vi "StateMachine_LIDAR.vi"() -> ()   [LabVIEW 2018]
uses:
  <vilib>/myRIO/Instrument Drivers/Onboard IO/DIO/typedefs/DIO Reference.ctl
  <vilib>/myRIO/Common/Instrument Driver Framework/Utilities/typedefs/myRIO Generic Hardware Reference.ctl
  <vilib>/myRIO/Common/Instrument Driver Framework/Utilities/typedefs/Hardware Version Enum.ctl
  <vilib>/myRIO/Common/Instrument Driver Framework/Utilities/typedefs/myRIO v1.0 Reference.ctl
  <vilib>/myRIO/Common/Instrument Driver Framework/Utilities/typedefs/Generic FPGA Reference.ctl
  <vilib>/myRIO/Common/Instrument Driver Framework/myRIO v1.0/DIO/typedefs/DIO Channels List.ctl
  <vilib>/myRIO/Common/Instrument Driver Framework/myRIO v1.0/DIO/typedefs/DIO Channels Enum.ctl
  <vilib>/userdefined/High Color/nirio_resource_hc.ctl
  enum_data_lidar.ctl
  <vilib>/myRIO/Common/Instrument Driver Framework/Utilities/vis/Is FPGA Ref Available.vi
  <vilib>/myRIO/Common/Instrument Driver Framework/myRIO v1.0/DIO/vis/myRIO v1.1 Open DIO.vi
  <vilib>/myRIO/Instrument Drivers/Onboard IO/DIO/vis/Write.vi
  <vilib>/myRIO/Common/Instrument Driver Framework/Utilities/vis/Validate Channels.vi
  <vilib>/myRIO/Common/Instrument Driver Framework/myRIO v1.0/DIO/vis/myRIO v1.0 Reserve DIO.vi
  <vilib>/myRIO/Common/Instrument Driver Framework/myRIO v1.0/Resource Manager/vis/myRIO v1.0 Reserve Channel List.vi
  <vilib>/myRIO/Common/Instrument Driver Framework/myRIO v1.0/DIO/vis/myRIO v1.0 Build MUX Configuration DIO.vi
  <vilib>/myRIO/Common/Instrument Driver Framework/myRIO v1.0/Resource Manager/vis/myRIO v1.0 Reserve Channel.vi
  <vilib>/myRIO/Common/Instrument Driver Framework/myRIO v1.0/Resource Manager/vis/myRIO v1.0 Unreserve Channel.vi
  <vilib>/myRIO/Common/Instrument Driver Framework/myRIO v1.0/Resource Manager/vis/myRIO v1.0 Create Configuration List.vi
  <vilib>/myRIO/Common/Instrument Driver Framework/myRIO v1.0/Resource Manager/vis/myRIO v1.0 Build Mutex Name.vi
  <vilib>/Utility/VariantDataType/GetNumericInfo.vi
  <vilib>/Utility/error.llb/Error Cluster From Error Code.vi
  <vilib>/myRIO/Common/Instrument Driver Framework/myRIO v1.0/myRIO v1.1 Open.vi
  <vilib>/myRIO/Common/Instrument Driver Framework/Utilities/vis/IO Manager.vi
  <vilib>/myRIO/Common/Instrument Driver Framework/Utilities/vis/Configuration Manager.vi
  <vilib>/myRIO/Common/Instrument Driver Framework/myRIO v1.0/Resource Manager/vis/myRIO v1.0 Configure IO.vi
  <vilib>/myRIO/Common/Instrument Driver Framework/myRIO v1.0/myRIO v1.0 Close.vi
  <vilib>/myRIO/Common/Instrument Driver Framework/myRIO v1.0/DIO/vis/myRIO v1.0 Write DIO.vi
  <vilib>/Instr/_visa.llb/VISA Configure Serial Port (Instr).vi
  <vilib>/myRIO/Express VI/Onboard IO/DO/DO Express VI.xnode
  <vilib>/myRIO/Instrument Drivers/Onboard IO/DIO/vis/myRIO DIO Open.xnode
  <vilib>/myRIO/Instrument Drivers/Onboard IO/DIO/DIO.lvlib
panel:
  out "Graphe XY":cluster{"X":dbl, "Y":dbl}[](graph)
  out "Data":cluster{"Angle":dbl, dbl}[](array[cluster])
  in  "Stop":bool
  out "NbPtsMesure":i32
  out "StartScan OK":bool
  out "Firmware":string
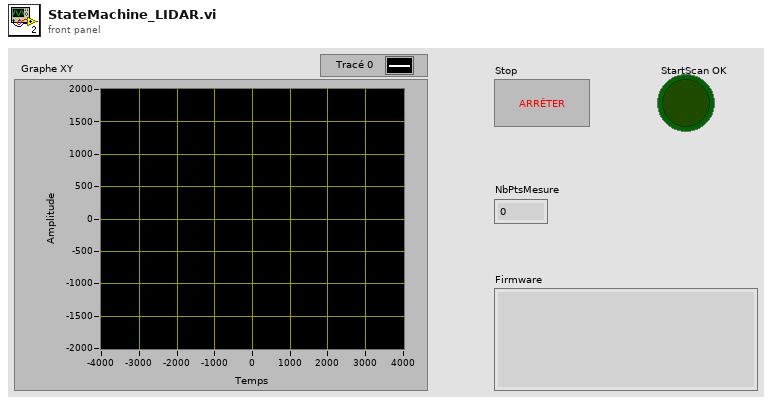
[diagram p1: front panel]
types:
  T1 = typedef "DIO.lvlib/DIO Reference.ctl" = cluster{"myRIO Reference":T2, "DIO Channels List":T6}
  T2 = typedef "myRIO Generic Hardware Reference.ctl" = cluster{"myRIO Model":T3, "myRIO Hardware Reference":T4}
  T3 = typedef "Hardware Version Enum.ctl" = enum16{"Unknown", "myRIO-1900", "myRIO-1950", "roboRIO", "NI ELVIS RIO CM", "ELVIS III"}
  T4 = typedef "myRIO v1.0 Reference.ctl" = cluster{"Generic FPGA Reference":T5, "Allow multiple opens":bool}
  T5 = typedef "Generic FPGA Reference.ctl" = refnum<k20>
  T6 = typedef "DIO Channels List.ctl" = T7[]
  T7 = typedef "DIO Channels Enum.ctl" = enum16{"Not Connected", "C/DIO0", "C/DIO1", "C/DIO2", "C/DIO3", "C/DIO4", "C/DIO5", "C/DIO6", "C/DIO7", "A/DIO0", "A/DIO1", "A/DIO2", "A/DIO3", "A/DIO4", "A/DIO5", "A/DIO6", "A/DIO7", "A/DIO8", "A/DIO9", "A/DIO10", "A/DIO11", "A/DIO12", "A/DIO13", "A/DIO14", "A/DIO15", "A/DIO16", "A/DIO17", "A/DIO18", "A/DIO19", "B/DIO0", "B/DIO1", "B/DIO2", "B/DIO3", "B/DIO4", "B/DIO5", "B/DIO6", "B/DIO7", "B/DIO8", "B/DIO9", "B/DIO10", "B/DIO11", "B/DIO12", "B/DIO13", "B/DIO14", "B/DIO15", "B/DIO16", "B/DIO17", "B/DIO18", "B/DIO19", "LED0", "LED1", "LED2", "LED3", "Button0", "DIO/DIO0", "DIO/DIO1", "DIO/DIO2", "DIO/DIO3", "DIO/DIO4", "DIO/DIO5", "DIO/DIO6", "DIO/DIO7", "DIO/DIO8", "DIO/DIO9", "SPI/CS0", "SPI/CS1", "SPI/CS2", "SPI/CS3", "LED RADIO (Green)", "LED RADIO (Red)", "LED COMM (Green)", "LED COMM (Red)", "LED MODE (Green)", "LED MODE (Red)"}
  T8 = typedef "nirio_resource_hc.ctl" = tag
  T9 = typedef "enum_data_lidar.ctl" = enum16{"Init", "Reset", "Start Scan", "Read Data", "Process Data", "Close"}
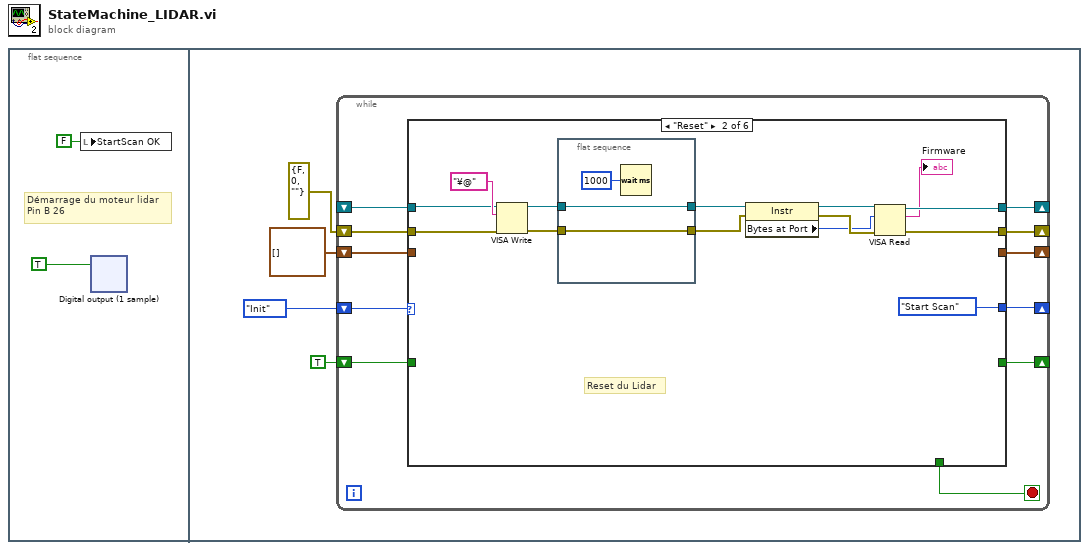
[diagram p0: block diagram]
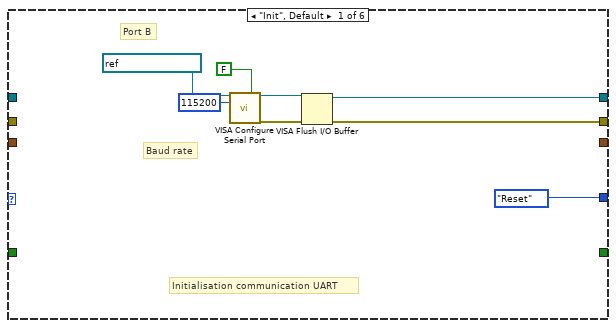
[diagram p2: hidden frame]
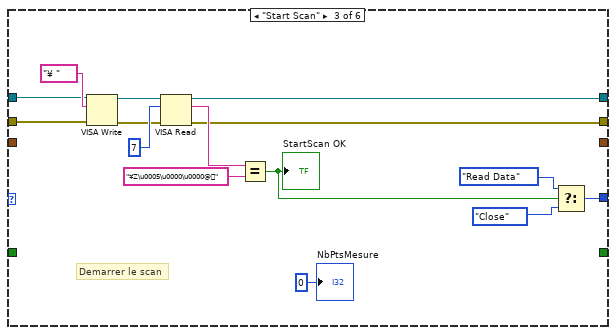
[diagram p3: hidden frame]
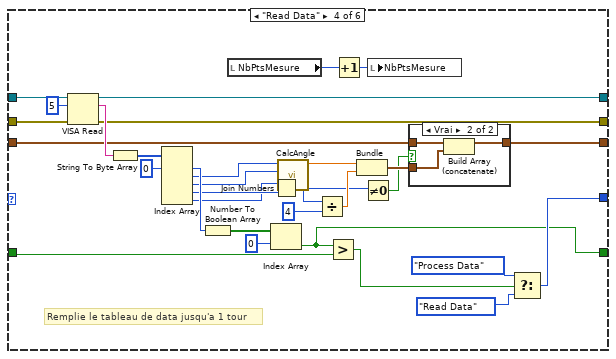
[diagram p4: hidden frame]
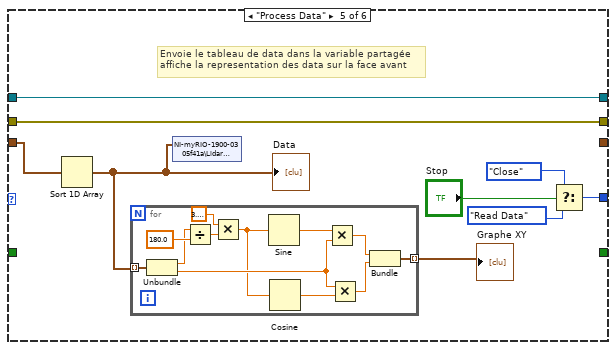
[diagram p6: hidden frame]
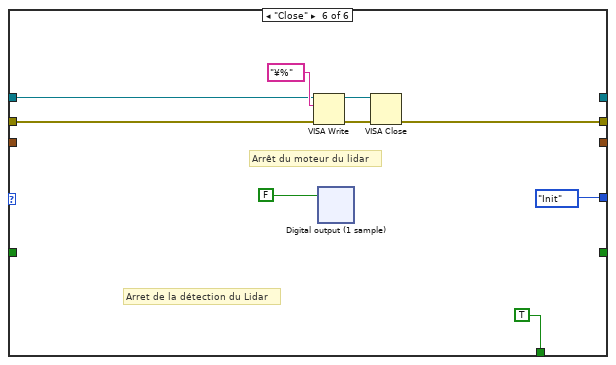
[diagram p7: hidden frame]
diagram:
  n1 = flat-sequence {
    frame #0 {
      # "Démarrage du moteur lidar\nPin B 26"
      n2 = local write "StartScan OK"(FALSE ("StartScan OK")) -> ()
      n3 = xnode "Digital output (1 sample)"("B/DIO13 (Pin 26)"=TRUE) -> ()  [unwired: 1 in, 1 out]
    }
    frame #1 {
      n4 = while {
        shift-right: [w47] -> _
        shift-left: enum_data_lidar."Init" ("Etats") -> [w52]
        shift-right: [w51] -> _
        shift-left: _ -> [w49]
        shift-right: [w50] -> _
        shift-left: errorcluster {"status"=FALSE, "code"=0, "source"=""} ("constante d'erreur") -> [w48]
        shift-right: [w44] -> _
        shift-left: TRUE -> [w45]
        shift-right: [w42] -> _
        shift-left: cluster{"Angle":dbl, dbl}[] [] -> [w43]
        stop <- w46 stop-if-true
        n5 = case shown="\"Reset\"" w52 {
          tunnel: [w55 w64 w84 w118 w136 _] -> w51
          tunnel: [w54 w63 w83 w119 w135 w152] -> w50
          tunnel: w49 -> [_ w71 w90 w123 w136 w154]
          tunnel: w48 -> [_ w70 w89 w122 w135 w153]
          tunnel: [enum_data_lidar."Reset" ("Etats") enum_data_lidar."Start Scan" ("Etats") w82 w117 w131 enum_data_lidar."Init" ("Etats")] -> w47
          tunnel: [_ _ _ _ _ TRUE] -> w46
          tunnel: w45 -> [_ _ _ w111 _ _]
          tunnel: [_ _ _ w112 _ _] -> w44
          tunnel: w43 -> [_ _ _ w108 w134 _]
          tunnel: [_ _ _ w107 _ _] -> w42
          frame "Init", Default {
            # "Baud rate"
            # "Port B"
            # "Initialisation communication UART"
            n6 = call-poly "VISA Configure Serial Port"("VISA resource name"=refnum<visa-resource-name> "ASRL2::INSTR", "Enable Termination\nChar (T)"=FALSE ("Enable Termination\nChar (T)"), "baud rate (9600)"=u32 115200) -> ("VISA resource name out"=w57:refnum<visa-resource-name>, "error out"=w56:errorcluster)  [unwired: 11 in]
            n7 = VISA Flush I/O Buffer(VISA resource name=w57, error in (no error)=w56) -> (VISA resource name out=w55:refnum<visa-resource-name>, error out=w54:errorcluster)  [unwired: 1 in]
          }
          frame "Reset" {
            # "Reset du Lidar"
            n8 = VISA Write(VISA resource name=w71, write buffer="¥@" ("Characters to Write"), error in (no error)=w70) -> (VISA resource name out=w74:refnum<visa-resource-name>, error out=w73:errorcluster)  [unwired: 1 out]
            n9 = flat-sequence {
              tunnel: w74 -> [w76]
              tunnel: w73 -> [w75]
              tunnel: [w76] -> w67
              tunnel: [w75] -> w66
              frame #0 {
                n10 = Wait (ms)(milliseconds to wait=u32 1000 ("attente (ms)")) -> ()  [unwired: 1 out]
              }
            }
            n11 = property class="Instr"(reference=w67, error in=w66) -> (reference out=w68:refnum<visa-resource-name>, error out=w69:errorcluster, "Bytes at Port"=w65:u32)
            n12 = VISA Read(VISA resource name=w68, byte count=w65, error in (no error)=w69) -> (VISA resource name out=w64:refnum<visa-resource-name>, read buffer=→"Firmware":string, error out=w63:errorcluster)  [unwired: 1 out]
          }
          frame "Start Scan" {
            # "Demarrer le scan"
            n13 = VISA Write(VISA resource name=w90, write buffer="¥ " ("Characters to Write"), error in (no error)=w89) -> (VISA resource name out=w87:refnum<visa-resource-name>, error out=w88:errorcluster)  [unwired: 1 out]
            n14 = VISA Read(VISA resource name=w87, byte count=u32 7 ("nombre d'octets"), error in (no error)=w88) -> (VISA resource name out=w84:refnum<visa-resource-name>, read buffer=w86:string, error out=w83:errorcluster)  [unwired: 1 out]
            n15 = Equal?(x=w86, y="¥Z\u0005\u0000\u0000@") -> (x = y?=w81:bool)
            "StartScan OK" <- w81
            n16 = Select(t=enum_data_lidar."Read Data" ("Etats"), s=w81, f=enum_data_lidar."Close" ("Etats")) -> (s? t:f=w82:T9)
            "NbPtsMesure" <- 0
          }
          frame "Read Data" {
            # "Remplie le tableau de data jusqu'a 1 tour"
            n17 = VISA Read(VISA resource name=w123, byte count=u32 5 ("nombre d'octets"), error in (no error)=w122) -> (VISA resource name out=w118:refnum<visa-resource-name>, read buffer=w120:string, error out=w119:errorcluster)  [unwired: 1 out]
            n18 = String To Byte Array(string=w120) -> (unsigned byte array=w110:u8[])
            n19 = Index Array(array=w110, index #1=0 ("indice")) -> (element #1=w106:u8, element #2=w105:u8, element #3=w104:u8, element #4=w103:u8, element #5=w102:u8)  [unwired: 4 in]
            n20 = Number To Boolean Array(number=w106) -> (Boolean array=w114:bool[])
            n21 = local read "NbPtsMesure"() -> (w116:i32)
            n22 = Index Array(array=w114, index=0 ("indice")) -> (element=w112:bool)
            n23 = Join Numbers(hi=w102, lo=w103) -> ((hi.lo)=w96:u16)
            n24 = call "CalcAngle.vi"("Octet 2"=w104, "Octet 1"=w105) -> ("Angle"=w101:dbl)  [unwired: 9 in]
            n25 = Divide(x=w96, y=u16 4) -> (x/y=w99:dbl)
            n26 = Greater?(x=w112, y=w111) -> (0:w97:bool)
            n27 = Increment(x=w116) -> (x+1=w115:i32)
            n28 = Bundle("Angle"=w101, w99) -> (w98:cluster{"Angle":dbl, dbl})  [unwired: 1 in]
            n29 = Not Equal To 0?(x=w96) -> (x != 0?=w95:bool)
            n30 = local write "NbPtsMesure"(w115) -> ()
            n31 = case shown="Vrai" w95 {
              tunnel: w108 -> [w124 w127]
              tunnel: [w124 w126] -> w107
              tunnel: w98 -> [_ w125]
              frame False {
              }
              frame True {
                n32 = Build Array (concatenate)(w127, w125) -> (w126:cluster{"Angle":dbl, dbl}[])
              }
            }
            n33 = Select(t=enum_data_lidar."Process Data" ("Etats"), s=w97, f=enum_data_lidar."Read Data" ("Etats")) -> (s? t:f=w117:T9)
          }
          frame "Process Data" {
            # "Envoie le tableau de data dans la variable partagée\naffiche la representation des data sur la face avant"
            n34 = Sort 1D Array(array=w134) -> (sorted array=w128:cluster{"Angle":dbl, dbl}[])
            "Data" <- w128
            n35 = for {
              tunnel: w128 -> [w148] mode=indexing
              tunnel: [w142] -> w133 mode=indexing
              n36 = Unbundle(w148) -> ("Angle"=w138:dbl, w146:dbl)
              n37 = Divide(x=w138, y=180.0) -> (x/y=w140:dbl)
              n38 = Multiply(x=3.141592653589793, y=w140) -> (x*y=w137:dbl)
              n39 = Sine(x=w137) -> (sin(x)=w147:dbl)
              n40 = Cosine(x=w137) -> (cos(x)=w145:dbl)
              n41 = Multiply(x=w147, y=w146) -> (x*y=w144:dbl)
              n42 = Multiply(x=w146, y=w145) -> (x*y=w143:dbl)
              n43 = Bundle(w144, w143) -> (w142:cluster{dbl, dbl})  [unwired: 1 in]
            }
            "Graphe XY" <- w133
            n44 = shared-variable "NI-myRIO-1900-0305f41a\\Lidar Library.lvlib\\Data"(w128) -> ()  [unwired: 1 in, 1 out]
            n45 = Select(t=enum_data_lidar."Close" ("Etats"), s="Stop", f=enum_data_lidar."Read Data" ("Etats")) -> (s? t:f=w131:T9)
          }
          frame "Close" {
            # "Arret de la détection du Lidar"
            # "Arrêt du moteur du lidar"
            n46 = VISA Write(VISA resource name=w154, write buffer="¥%" ("Characters to Write"), error in (no error)=w153) -> (VISA resource name out=w155:refnum<visa-resource-name>, error out=w156:errorcluster)  [unwired: 1 out]
            n47 = xnode "Digital output (1 sample)"("B/DIO13 (Pin 26)"=FALSE) -> ()  [unwired: 1 in, 1 out]
            n48 = VISA Close(VISA resource name=w155, error in (no error)=w156) -> (error out=w152:errorcluster)
          }
        }
      }
    }
  }
